vi "Ecrire_alarmes_fichier_rapport_profil.vi"(1 "Alarme haute (°C)":dbl, 2 "Alarme basse (°C)":dbl, 3 "Nom Regulateur":string, 4 "Fichier rapport":path) -> ()   [LabVIEW 2022 SP3]
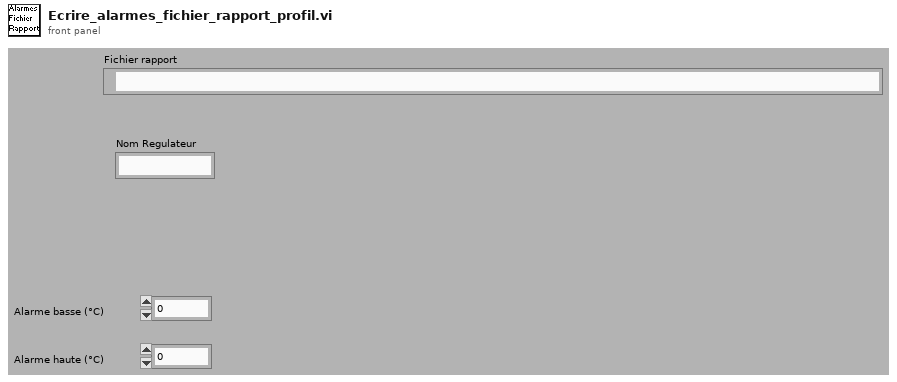
[diagram p1: front panel]
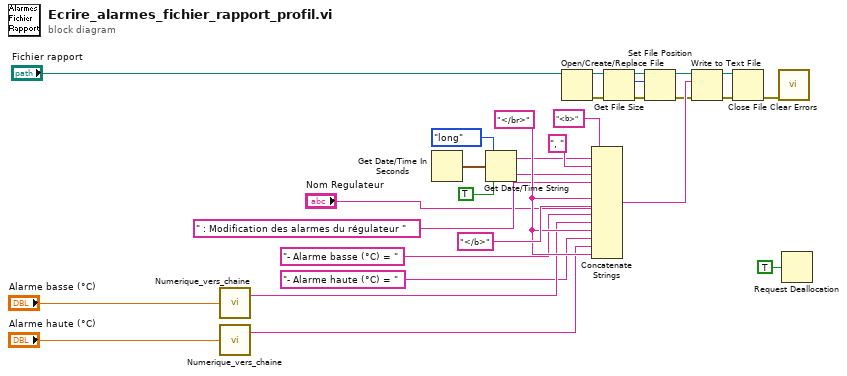
[diagram p0: block diagram]
diagram:
  w28 = "</br>" ("chaîne")
  n1 = call "Numerique_vers_chaine.vi"("Valeur numérique"="Alarme basse (°C)") -> ("Chaine sans zéros inutiles"=w16:string)  [unwired: 1 out]
  n2 = call "Numerique_vers_chaine.vi"("Valeur numérique"="Alarme haute (°C)") -> ("Chaine sans zéros inutiles"=w17:string)  [unwired: 1 out]
  n3 = Get Date/Time In Seconds() -> (seconds since 1Jan1904=w7:timestamp)
  n4 = Get Date/Time String(date format (0)=enum16{"short", "long", "abbreviated"}."long" ("format de date (0)"), seconds (now)=w7, want seconds? (F)=TRUE ("secondes ? (F)")) -> (date string=w10:string, time string=w12:string)
  n5 = Open/Create/Replace File(file path (use dialog)="Fichier rapport") -> (refnum out=w23:refnum<file>, error out=w24:errorcluster)  [unwired: 5 in, 1 out]
  n6 = Concatenate Strings("<b>" ("chaîne"), w10, ", " ("chaîne"), w12, " : Modification des alarmes du régulateur " ("chaîne"), "Nom Regulateur", w28, "</b>" ("chaîne"), "- Alarme basse (°C) = ", w16, w28, "- Alarme haute (°C) = ", w17, w28) -> (w22:string)
  n7 = Get File Size(file=w23, error in=w24) -> (refnum out=w27:refnum<file>, size (in bytes)=w26:i64, 0:w25:errorcluster)
  n8 = Set File Position(offset (in bytes) (0)=w26, refnum=w27, error in=w25) -> (refnum out=w19:refnum<file>, error out=w18:errorcluster)  [unwired: 1 in]
  n9 = Write to Text File(file (use dialog)=w19, text=w22, error in=w18) -> (refnum out=w20:refnum<file>, error out=w21:errorcluster)  [unwired: 1 in, 1 out]
  n10 = Close File(refnum=w20, error in=w21) -> (error out=w3:errorcluster)  [unwired: 1 out]
  n11 = call <vilib>:"Clear Errors.vi"("error in (no error)"=w3) -> ()  [unwired: 5 in, 2 out]
  n12 = Request Deallocation(TRUE ("flag")) -> ()
